vi "check Resource Array-PPS.vi"(8 "error in":errorcluster, 11 "Resource names":string[](array[string])) -> (0 "error out":errorcluster, 1 "Slave resource names":string[](array[string]), 2 "Single/Master resouce names":string, 3 "Single or ganged configuration":bool)   [LabVIEW 2021]
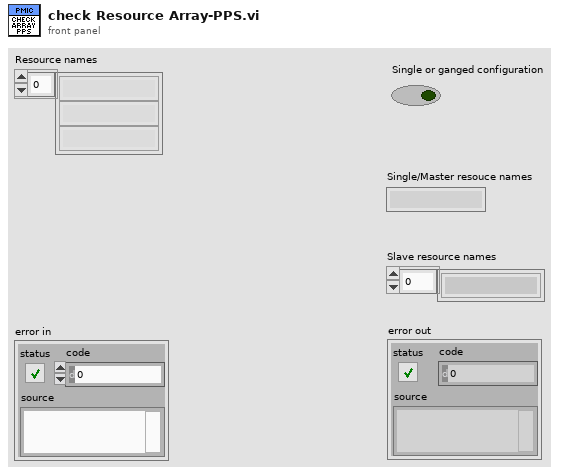
[diagram p1: front panel]
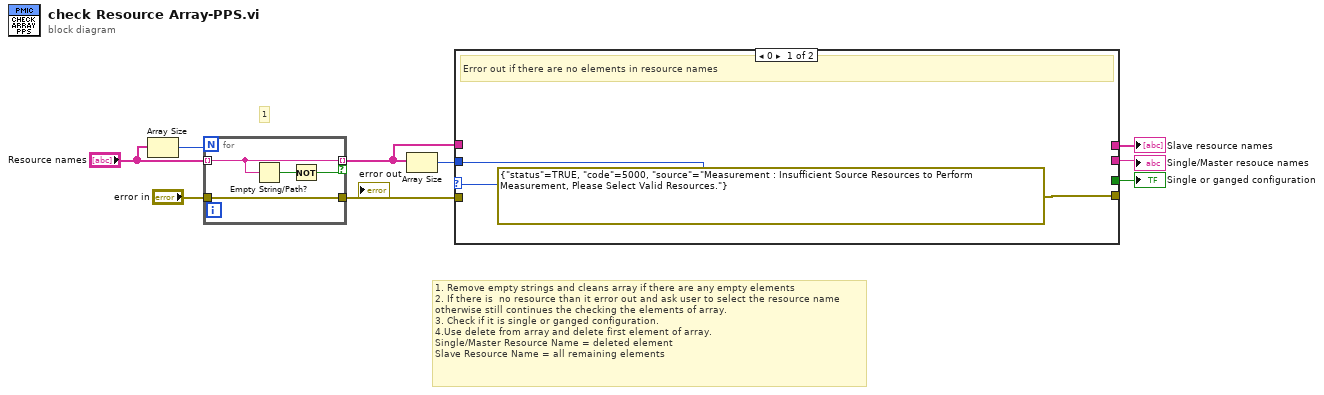
[diagram p0: block diagram]
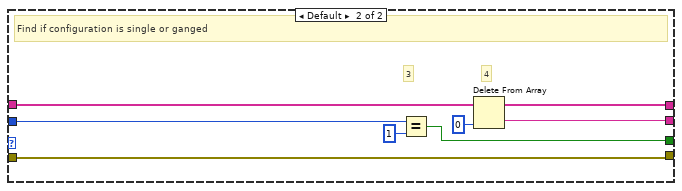
[diagram p2: hidden frame]
diagram:
  # "1"
  # "1. Remove empty strings and cleans array if there are any empty elements\n2. If there is  no resource than it error out and ask user to select the resource name\notherwise still continues the checking the elements of array.\n3. Check if it is single or ganged configuration.\n4.Use delete from array and delete first element of array.\nSingle/Master Resource Name = deleted element\nSlave Resource Name = all remaining elements"
  n1 = Array Size(array="Resource names") -> (size(s)=w9:i32)
  n2 = for {
    N: w9 -> [_]
    tunnel: "Resource names" -> [w10] mode=indexing
    tunnel: "error in" -> [w13]
    tunnel: [w13] -> w1
    tunnel: [w10] -> w5 mode=indexing if=w11
    n3 = Empty String/Path?(string/path=w10) -> (empty?=w12:bool)
    n4 = Not(x=w12) -> (.not. x?=w11:bool)
  }
  n5 = Array Size(array=w5) -> (size(s)=w2:i32)
  n6 = case shown="0" w2 {
    tunnel: w2 -> [_ w22]
    tunnel: [_ w20] -> w6
    tunnel: w5 -> [_ w19]
    tunnel: [_ w17] -> w4
    tunnel: [_ w16] -> w3
    tunnel: w1 -> [_ w15]
    tunnel: [errorcluster {"status"=TRUE, "code"=5000, "source"="Measurement : Insufficient Source Resources to Perform Measurement, Please Select Valid Resources."} ("error constant") w15] -> _
    frame 0 {
      # "Error out if there are no elements in resource names"
    }
    frame Default {
      # "4"
      # "3"
      # "Find if configuration is single or ganged"
      n7 = Equal?(x=w22, y=1) -> (x = y?=w20:bool)
      n8 = Delete From Array(array=w19, index=0) -> (deleted portion=w16:string, array with subset deleted=w17:string[])  [unwired: 1 in]
    }
  }
  "Single or ganged configuration" <- w6
  "Single/Master resouce names" <- w3
  "Slave resource names" <- w4
